vi "Create MQTT Client.vi"(5 "Client in":refnum<class "Client.lvclass">, 6 "Enable Mutex ? (F)":bool, 8 "error in (no error)":errorcluster, 10 "Connection Configuration":refnum<class "Connection.lvclass">, 11 "ID (empty:generate new)":string) -> (0 "error out":errorcluster, 3 "Client out":refnum<class "Client.lvclass">)   [LabVIEW 2013, in "MQTT Client.lvlib" / "Client.lvclass"]
uses:
  Client.lvclass
  <vilib>/LabVIEW Open Source Project/Connection/Connection/Connection.lvclass
  <vilib>/LabVIEW Open Source Project/MQTT Control Packets/Control Packets/CONNACK/Connect Return Code -- enum.ctl
  <vilib>/LabVIEW Open Source Project/MQTT Control Packets/Control Packets/PUBLISH/PUBLISH.lvclass
  <vilib>/LabVIEW Open Source Project/MQTT Connection/MQTT_Base/Base Class/MQTT_Base.lvclass/MQTT_Base.ctl
  Client.lvclass/Client.ctl
  <vilib>/LabVIEW Open Source Project/OpenSerializer/Serializer.FlattenedString/Serializer.FlattenedString.lvclass
  <vilib>/LabVIEW Open Source Project/OpenSerializer/Serializer/Serializer.lvclass
  <vilib>/LabVIEW Open Source Project/MQTT Control Packets/Control Packets/ControlPacket/ControlPacket.lvclass
  <vilib>/LabVIEW Open Source Project/MQTT Control Packets/Control Packets/CONNACK/CONNACK.lvclass
  <vilib>/LabVIEW Open Source Project/MQTT Connection/MQTT_Base/Base Class/MQTT_Base.lvclass
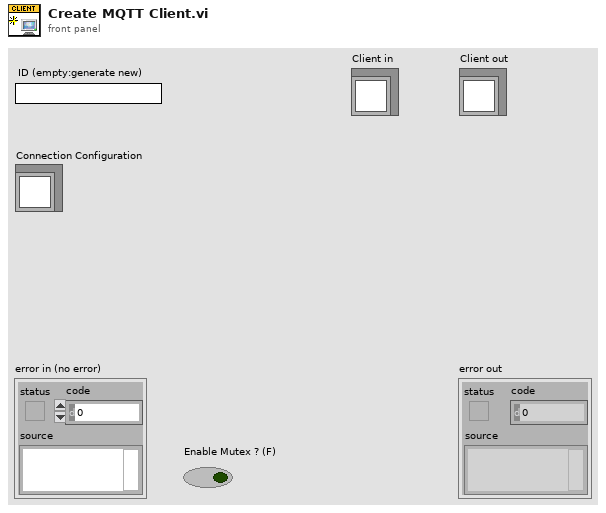
[diagram p1: front panel]
types:
  T1 = typedef "MQTT_Control_Packets.lvlib/CONNACK.lvclass/Connect Return Code -- enum.ctl" = enum16{"Connection accepted", "Unacceptable protocol version", "Identifier Rejected", "Server Unavailable", "Bad Username or Password", "Not Authorized"}
  T2 = typedef "Semaphore RefNum" = refnum<k1>
  T3 = cluster{"Connection Status":refnum<user-event>, "Connected":refnum<user-event>, "Application Message":refnum<user-event>}
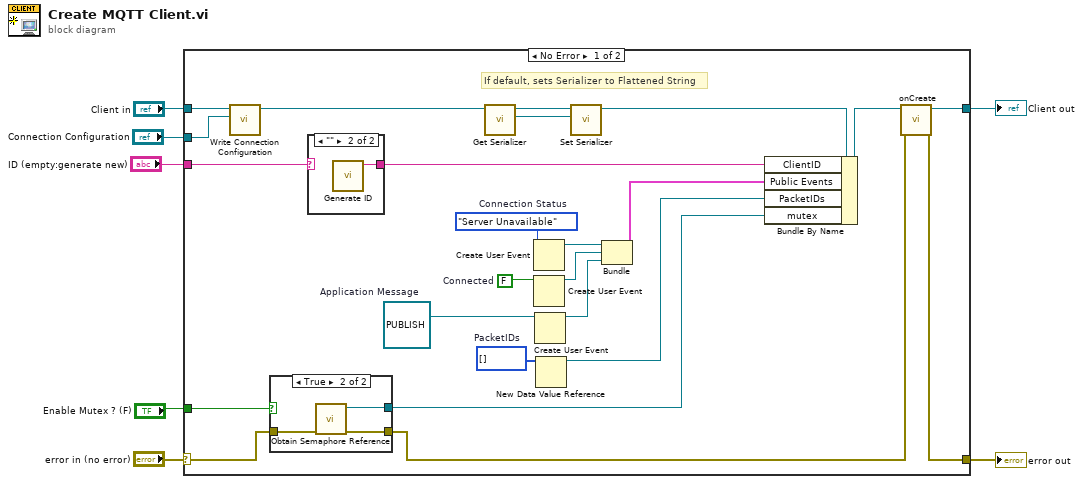
[diagram p0: block diagram]
diagram:
  n1 = case shown="No Error" "error in (no error)" {
    selector: "error in (no error)" -> [w9 w39]
    tunnel: [w27 w39] -> w3
    tunnel: [w28 w38] -> w4
    tunnel: "Client in" -> [w14 w38]
    tunnel: "ID (empty:generate new)" -> [w31 _]
    tunnel: "Connection Configuration" -> [w12 _]
    tunnel: "Enable Mutex ? (F)" -> [w11 _]
    frame No Error {
      w19 = u16[] []  # PacketIDs
      w21 = refnum<class "PUBLISH.lvclass"> refnum  # Application Message
      w22 = FALSE  # Connected
      w24 = Connect_Return_Code_--_enum."Server Unavailable"  # Connection Status
      # "If default, sets Serializer to Flattened String"
      n2 = call <vilib>:"Write Connection Configuration.vi"("Connection Configuration"=w12, "MQTT_Base in"=w14) -> ("MQTT_Base out"=w13:refnum<class "Client.lvclass">)  [unwired: 8 in, 1 out]
      n3 = case shown="True" w11 {
        tunnel: [_ w35] -> w10
        tunnel: w9 -> [w32 w34]
        tunnel: [w32 w33] -> w8
        frame False {
        }
        frame True {
          n4 = call <vilib>:"Obtain Semaphore Reference.vi"("error in (no error)"=w34) -> ("error out"=w33:errorcluster, "semaphore"=w35:T2)  [unwired: 4 in, 1 out]
        }
      }
      n5 = case shown="\"\"" w31 {
        selector: w31 -> [w36 _]
        tunnel: [w36 w37] -> w30
        frame Default {
        }
        frame "" {
          n6 = call <vilib>:"Generate ID.vi"() -> ("ID"=w37:string)  [unwired: 11 in]
        }
      }
      n7 = call <vilib>:"Get Serializer.vi"("MQTT_Base"=w13) -> ("Serializer"=w15:refnum<class "Serializer.lvclass">, "MQTT_Base out"=w17:refnum<class "Client.lvclass">)  [unwired: 8 in, 1 out]
      n8 = Create User Event(user event datatype=w24) -> (user event=w26:refnum<user-event>)  [unwired: 1 in, 1 out]
      n9 = Create User Event(user event datatype=w22) -> (user event=w23:refnum<user-event>)  [unwired: 1 in, 1 out]
      n10 = Create User Event(user event datatype=w21) -> (user event=w20:refnum<user-event>)  [unwired: 1 in, 1 out]
      n11 = New Data Value Reference(data value=w19) -> (data value reference=w18:refnum<data-value>)  [unwired: 1 in, 1 out]
      n12 = call <vilib>:"Set Serializer.vi"("Serializer (default: Flattened String)"=w15, "MQTT_Base"=w17) -> ("MQTT_Base out"=w16:refnum<class "Client.lvclass">)  [unwired: 8 in, 1 out]
      n13 = Bundle("Connection Status"=w26, "Connected"=w23, "Application Message"=w20) -> (w25:T3)  [unwired: 1 in]
      n14 = Bundle By Name(cluster=w16, "ClientID"=w30, "Public Events"=w25, "PacketIDs"=w18, "mutex"=w10) -> (w29:refnum<class "Client.lvclass">)
      n15 = call-dynamic "onCreate.vi"("error in (no error)"=w8, "Client in"=w29) -> ("error out"=w27:errorcluster, "Client out"=w28:refnum<class "Client.lvclass">)  [unwired: 8 in]
    }
    frame Error {
    }
  }
  "error out" <- w3
  "Client out" <- w4
